vi "DAC Init Results.vi"(8 "error in":errorcluster, 9 "Log Details?":bool, 10 "tdms file":refnum<k34>, 11 "DAC Pressure Scan in":refnum<class "DAC Pressure Scan.lvclass">) -> (0 "error out":errorcluster, 2 "tdms file out":refnum<k34>)   [LabVIEW 2019, in "DAC.lvlib" / "DAC Pressure Scan.lvclass"]
uses:
  DAC Pressure Scan.lvclass
  C:/Users/wg/Documents/LV_Projects/test-stand/App/DAC/DAC.lvclass
  DAC.lvclass/DAC.ctl
  DAC Pressure Scan.lvclass/DAC Pressure Scan.ctl
  DAC.lvclass
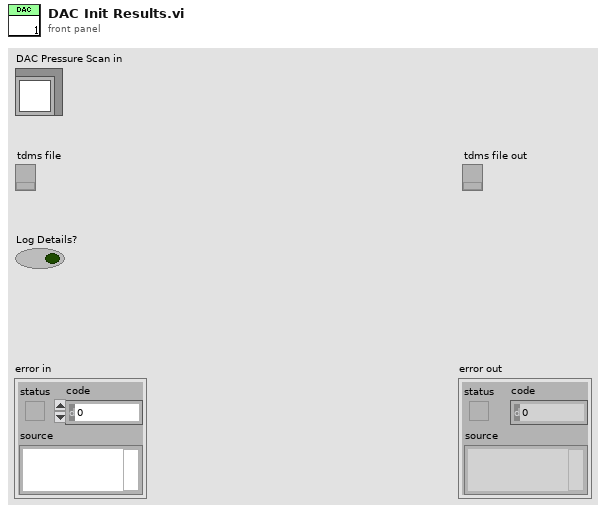
[diagram p1: front panel]
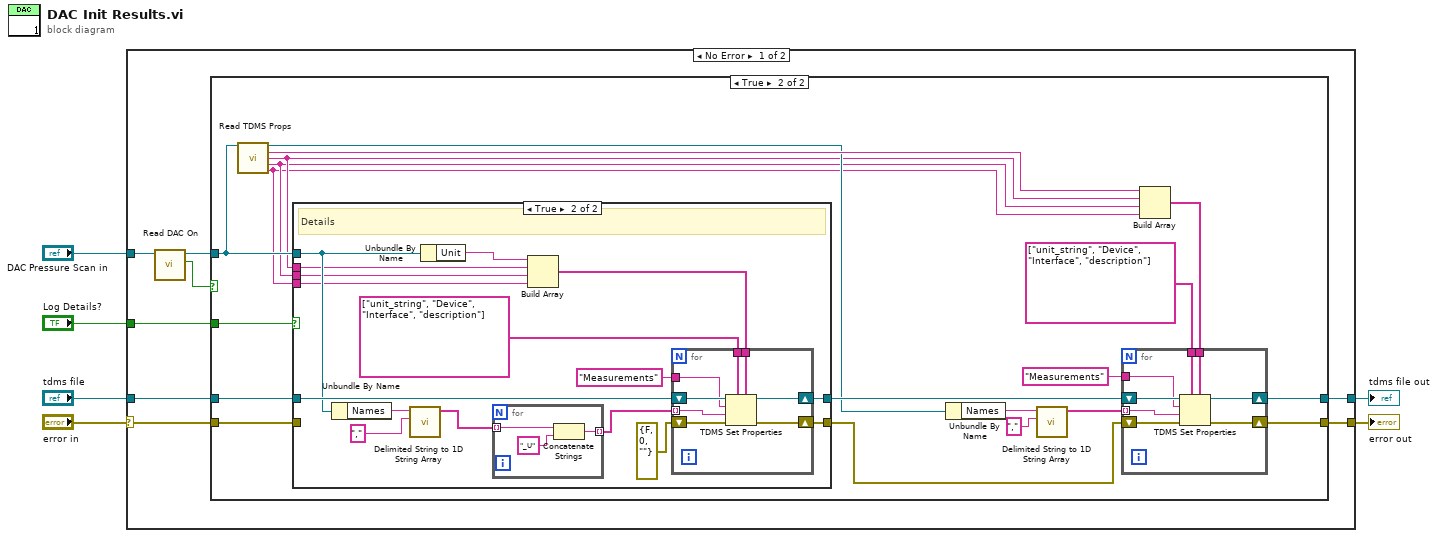
[diagram p0: block diagram]
diagram:
  n1 = case shown="No Error" "error in" {
    selector: "error in" -> [w8 w74]
    tunnel: [w12 w74] -> w3
    tunnel: "DAC Pressure Scan in" -> [w11 _]
    tunnel: "tdms file" -> [w14 w73]
    tunnel: [w13 w73] -> w2
    tunnel: "Log Details?" -> [w7 _]
    frame No Error {
      n2 = call "Read DAC On.vi"("DAC in"=w11) -> ("DAC On"=w9:bool, "DAC out"=w10:refnum<class "DAC Pressure Scan.lvclass">)  [unwired: 8 in, 1 out]
      n3 = case shown="True" w9 {
        tunnel: w14 -> [w16 w29]
        tunnel: [w16 w35] -> w13
        tunnel: [w15 w34] -> w12
        tunnel: w10 -> [_ w23]
        tunnel: w8 -> [w15 w25]
        tunnel: w7 -> [_ w30]
        frame False {
        }
        frame True {
          n4 = call "Read TDMS Props.vi"("DAC in"=w23) -> ("DAC out"=w22:refnum<class "DAC Pressure Scan.lvclass">, "Result Unit"=w24:string, "DAC Device"=w21:string, "DAC IO"=w20:string, "DAC Description"=w19:string)  [unwired: 10 in]
          n5 = case shown="True" w30 {
            tunnel: w29 -> [w37 w51]
            tunnel: [w37 w50] -> w28
            tunnel: w23 -> [_ w41]
            tunnel: [w36 w47] -> w26
            tunnel: w25 -> [w36 _]
            tunnel: w21 -> [_ w40]
            tunnel: w20 -> [_ w39]
            tunnel: w19 -> [_ w38]
            frame False {
            }
            frame True {
              # "Details"
              n6 = Unbundle By Name(w41) -> ("Names"=w52:string)
              n7 = call <vilib>:"Delimited String to 1D String Array.vi"("delimiter"=",", "delimited string"=w52) -> ("string array"=w49:string[])  [unwired: 9 in]
              n8 = Unbundle By Name(w41) -> ("Unit"=w44:string)
              n9 = for {
                tunnel: w49 -> [w56] mode=indexing
                tunnel: [w54] -> w45 mode=indexing
                n10 = Concatenate Strings(w56, "_U" ("string")) -> (w54:string)
              }
              n11 = Build Array(w44, w40, w39, w38) -> (w42:string[])
              n12 = for {
                tunnel: string[] ["unit_string", "Device", "Interface", "description"] ("property names") -> [w63]
                tunnel: w42 -> [w62]
                shift-right: [w61] -> w50
                shift-left: w51 -> [w64]
                tunnel: "Measurements" ("group name in (Untitled)") -> [w59]
                shift-right: [w60] -> w47
                shift-left: errorcluster {"status"=FALSE, "code"=0, "source"=""} ("error out") -> [w58]
                tunnel: w45 -> [w57] mode=indexing
                n13 = TDMS Set Properties(5:w62, 7:w63, 8:w58, 9:w57, 10:w59, 11:w64) -> (0:w60:errorcluster, 3:w61:refnum<k34>)  [unwired: 2 out]
              }
            }
          }
          n14 = Unbundle By Name(w22) -> ("Names"=w31:string)
          n15 = call <vilib>:"Delimited String to 1D String Array.vi"("delimiter"=",", "delimited string"=w31) -> ("string array"=w33:string[])  [unwired: 9 in]
          n16 = Build Array(w24, w21, w20, w19) -> (w17:string[])
          n17 = for {
            tunnel: w33 -> [w71] mode=indexing
            tunnel: string[] ["unit_string", "Device", "Interface", "description"] ("property names") -> [w70]
            tunnel: w17 -> [w69]
            shift-right: [w68] -> w35
            shift-left: w28 -> [w72]
            tunnel: "Measurements" ("group name in (Untitled)") -> [w66]
            shift-right: [w67] -> w34
            shift-left: w26 -> [w65]
            n18 = TDMS Set Properties(5:w69, 7:w70, 8:w65, 9:w71, 10:w66, 11:w72) -> (0:w67:errorcluster, 3:w68:refnum<k34>)  [unwired: 2 out]
          }
        }
      }
    }
    frame Error {
    }
  }
  "error out" <- w3
  "tdms file out" <- w2
